vi "RemoteVI Window Info.vi"(0 "hWnd":u64, 5 "frame origin":cluster{"x":i32, "y":i32}, 7 "panel enabled?":bool=TRUE, 9 "active":u64, 11 "error in":errorcluster) -> (4 "window":T1, 15 "error out":errorcluster)   [LabVIEW 2020, in "RemoteVI.lvlib"]
doc: "Everything the windows message and the input routing need about one listed window (docs\\protocol.md section 7): id = hWnd; title = its caption as a JSON string literal (user32 GetWindowTextW.vi + RemoteVI JSON String.vi) - a window without a caption gets its OWNER's caption (a LabVIEW Two Button Dialog has none and is owned by LabVIEW's hidden frame window, caption LabVIEW; measured on LabVIEW 2025), and LabVIEW when that is empty too; x, y, w, h = its client area (RemoteVI Frame Rect.vi) relative to the main frame's origin on screen; modal = the published panel is disabled; active = it is the active window of its thread; closable = its style has WS_SYSMENU (0x80000, the title bar's close box); sx, sy = its client-area origin on screen; class = its window class (#32770 is a native Windows dialog). Win32 calls only, no VI Server, so it works while a dialog's modal loop holds LabVIEW's UI thread."
uses:
  RemoteVI.lvlib
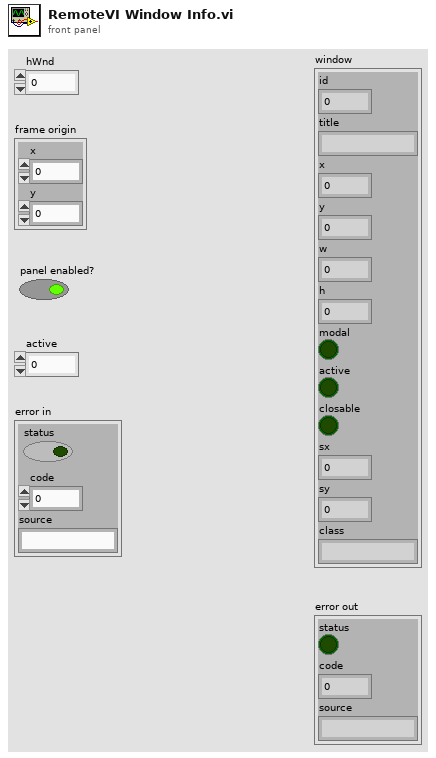
[diagram p1: front panel]
types:
  T1 = cluster{"id":u64, "title":string, "x":i32, "y":i32, "w":i32, "h":i32, "modal":bool, "active":bool, "closable":bool, "sx":i32, "sy":i32, "class":string}
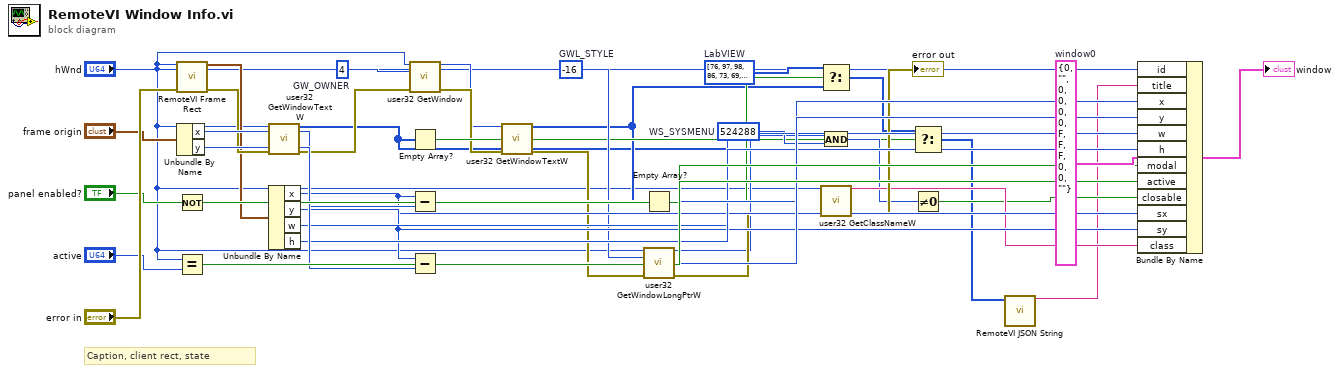
[diagram p0: block diagram]
diagram:
  w39 = T1 {"id"=0, "title"="", "x"=0, "y"=0, "w"=0, "h"=0, "modal"=FALSE, "active"=FALSE, "closable"=FALSE, "sx"=0, "sy"=0, "class"=""}  # window0
  w24 = i64 524288  # WS_SYSMENU
  w21 = -16  # GWL_STYLE
  w15 = u16[] [76, 97, 98, 86, 73, 69, 87]  # LabVIEW
  w10 = u32 4  # GW_OWNER
  # "Caption, client rect, state"
  n1 = call "RemoteVI Frame Rect.vi"("hWnd"="hWnd", "error in"="error in") -> ("rect"=w6:cluster{"x":i32, "y":i32, "w":i32, "h":i32}, "error out"=w7:errorcluster)  [unwired: 12 in]
  n2 = Unbundle By Name("frame origin") -> ("x"=w33:i32, "y"=w34:i32)
  n3 = Not(x="panel enabled?") -> (.not. x?=w37:bool)
  n4 = Equal?(x="hWnd", y="active") -> (x = y?=w38:bool)
  n5 = call "user32 GetWindowTextW.vi"("hWnd"="hWnd", "error in"=w7) -> ("text"=w8:u16[], "error out"=w9:errorcluster)  [unwired: 11 in, 1 out]
  n6 = Unbundle By Name(w6) -> ("x"=w29:i32, "y"=w30:i32, "w"=w31:i32, "h"=w32:i32)
  n7 = call "user32 GetWindow.vi"("hWnd"="hWnd", "uCmd"=w10, "error in"=w9) -> ("window"=w11:u64, "error out"=w12:errorcluster)  [unwired: 11 in]
  n8 = Empty Array?(array=w8) -> (empty?=w18:bool)
  n9 = Subtract(x=w29, y=w33) -> (x-y=w35:i32)
  n10 = Subtract(x=w30, y=w34) -> (x-y=w36:i32)
  n11 = call "user32 GetWindowTextW.vi"("hWnd"=w11, "error in"=w12) -> ("text"=w13:u16[], "error out"=w14:errorcluster)  [unwired: 11 in, 1 out]
  n12 = Empty Array?(array=w13) -> (empty?=w16:bool)
  n13 = call "user32 GetWindowLongPtrW.vi"("hWnd"="hWnd", "nIndex"=w21, "error in"=w14) -> ("return value"=w22:i64, "error out"=w23:errorcluster)  [unwired: 11 in]
  n14 = Select(t=w15, s=w16, f=w13) -> (s? t:f=w17:u16[])
  n15 = And(x=w22, y=w24) -> (x .and. y?=w25:i64)
  n16 = call "user32 GetClassNameW.vi"("hWnd"="hWnd", "error in"=w23) -> ("class name"=w27:string, "error out"=→"error out":errorcluster)  [unwired: 11 in, 1 out]
  n17 = Select(t=w17, s=w18, f=w8) -> (s? t:f=w19:u16[])
  n18 = Not Equal To 0?(x=w25) -> (x != 0?=w26:bool)
  n19 = call "RemoteVI JSON String.vi"("text"=w19) -> ("json"=w20:string)  [unwired: 14 in]
  n20 = Bundle By Name(cluster=w39, "id"="hWnd", "title"=w20, "x"=w35, "y"=w36, "w"=w31, "h"=w32, "modal"=w37, "active"=w38, "closable"=w26, "sx"=w29, "sy"=w30, "class"=w27) -> (→"window":T1)
